vi "talking tom.vi"() -> ()   [LabVIEW 2018]
panel:
  out "Waveform Chart":waveform(dbl)(graph)
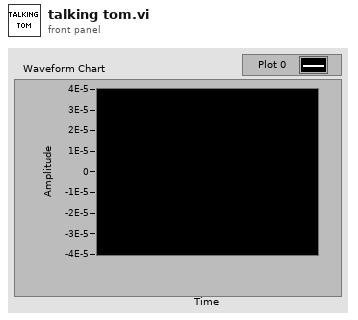
[diagram p1: front panel]
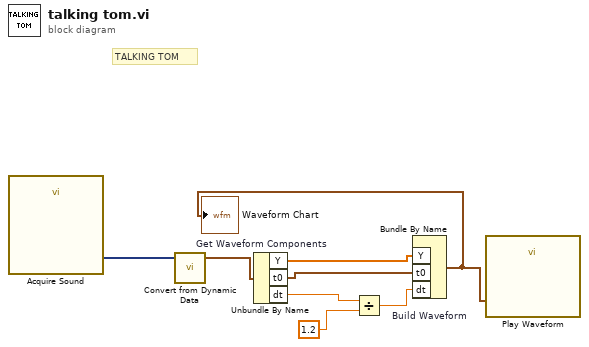
[diagram p0: block diagram]
diagram:
  # "TALKING TOM"
  n1 = call "Acquire Sound"() -> ("Data"=w8:dynamicdata)  [unwired: 18 in, 1 out]
  n2 = call "Convert from Dynamic Data"("Dynamic Data Type"=w8) -> ("Waveform"=w7:waveform(dbl))  [unwired: 3 in]
  n3 = Unbundle By Name "Get Waveform Components"(w7) -> ("Y"=w4:dbl[], "t0"=w3:timestamp, "dt"=w6:dbl)
  n4 = Divide(x=w6, y=1.2) -> (x/y=w2:dbl)
  n5 = Bundle By Name "Build Waveform"("Y"=w4, "t0"=w3, "dt"=w2) -> (w1:waveform(dbl))  [unwired: 1 in]
  "Waveform Chart" <- w1
  n6 = call "Play Waveform"("Data"=w1) -> ()  [unwired: 18 in, 1 out]
